vi "MergeSort.vi"(8 "Sort VI":T1, 11 "ArrayPanelRefs":refnum<data-value>[](array[refnum])) -> (3 "Sorted ArrayPanelRefs":refnum<data-value>[](array[refnum]))   [LabVIEW 2020, in "OOPanel.lvlib" / "ArrayManager.lvclass"]
uses:
  ArrayManager.lvclass
  ArrayPanel/ArrayPanel.lvclass
  Sort VI Type.ctl
  Panel/Panel.lvclass
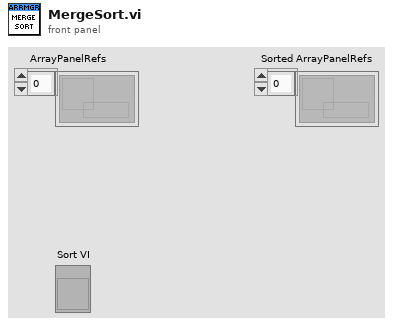
[diagram p1: front panel]
types:
  T1 = typedef "OOPanel.lvlib/ArrayManager.lvclass/Sort VI Type.ctl" = refnum<vi>
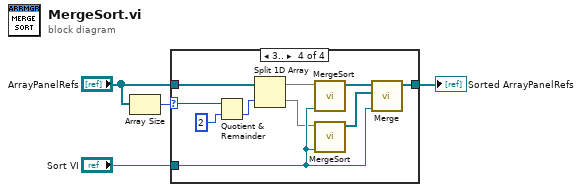
[diagram p0: block diagram]
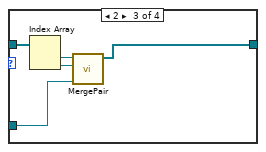
[diagram p4: hidden frame]
diagram:
  n1 = Array Size(array="ArrayPanelRefs") -> (size(s)=w4:i32)
  n2 = case shown="3.." w4 {
    selector: w4 -> [_ _ _ w19]
    tunnel: "ArrayPanelRefs" -> [w5 w6 w11 w18]
    tunnel: "Sort VI" -> [_ _ w8 w21]
    tunnel: [w5 w6 w7 w12] -> w1
    frame ..-1 {
    }
    frame 0, 1 {
    }
    frame 2 {
      n3 = Index Array(array=w11) -> (element #1=w10:refnum<data-value>, element #2=w9:refnum<data-value>)  [unwired: 2 in]
      n4 = call "MergePair.vi"("Sort VI"=w8, "B"=w9, "A"=w10) -> ("Merged"=w7:refnum<data-value>[])  [unwired: 8 in]
    }
    frame 3.. {
      n5 = Quotient & Remainder(x=w19, y=2) -> (floor(x/y)=w17:i32)  [unwired: 1 out]
      n6 = Split 1D Array(array=w18, index=w17) -> (first subarray=w15:refnum<data-value>[], second subarray=w16:refnum<data-value>[])
      n7 = call "MergeSort.vi"("Sort VI"=w21, "ArrayPanelRefs"=w15) -> ("Sorted ArrayPanelRefs"=w14:refnum<data-value>[])  [unwired: 9 in]
      n8 = call "MergeSort.vi"("Sort VI"=w21, "ArrayPanelRefs"=w16) -> ("Sorted ArrayPanelRefs"=w13:refnum<data-value>[])  [unwired: 9 in]
      n9 = call "Merge.vi"("Sort VI"=w21, "B"=w13, "A"=w14) -> ("Merged"=w12:refnum<data-value>[])  [unwired: 8 in]
    }
  }
  "Sorted ArrayPanelRefs" <- w1
